vi "Create Palettes for VIs in Folder.vi"(5 "Create palettes for LLBs (F)":bool, 6 "Filter Options":T1={"Exclude Dir Name pattern(s)"="^_", "Exclude LLB Name pattern(s)"="^_", "Exclude VI Name pattern(s)"="^_"}, 7 "Palette Icon":picture, 8 "error in":errorcluster, 9 "Save sub-palettes in sub-folders (F)":bool, 10 "Folder or LLB Path":path, 11 "Palette File Path (empty)":path) -> (0 "error out":errorcluster, 2 "All Palette File Paths":path[](array[path]), 3 "Palette File Path out":path)   [LabVIEW 2014, in "VIHelpeksAPI.lvlib"]
doc: "The VI creates palette files for VIs in a folder. It creates a palette for every sub-folder and LLB beneath the given folder recursively.\n\n<b>Palette icons</b>\nFor the given folder and all sub-folders beneath it, the VI looks for an image file to use as an icon for the respective palette. A folder's icon file can be one of the following:\n(1) A file with the same name as the folder and a <b>.png</b> extension that resides in the folder's parent directory.\n(2) A file with the <b>dir_icon.png</b> name that resides inside the folder itself.\nIf neither of these icon files is found, a default icon is applied to the respective palette.\nThe icon of the top-level palette can be defined explicitly in the <b>Palette Icon</b> input terminal.\n\n\n::: VI Helpeks :::\nCopyright (c) 2000-2026 Konstantin Shifershteyn. All rights reserved."
uses:
  VIHelpeksAPI.lvlib
panel:
  # "VI Helpeks\nCopyright (c) 2012-2026 Konstantin Shifershteyn"
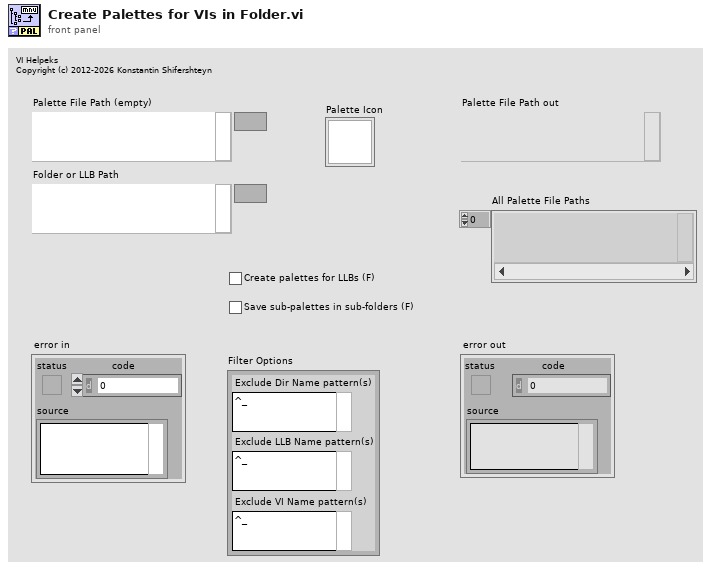
[diagram p1: front panel]
types:
  T1 = cluster{"Exclude Dir Name pattern(s)":string, "Exclude LLB Name pattern(s)":string, "Exclude VI Name pattern(s)":string}
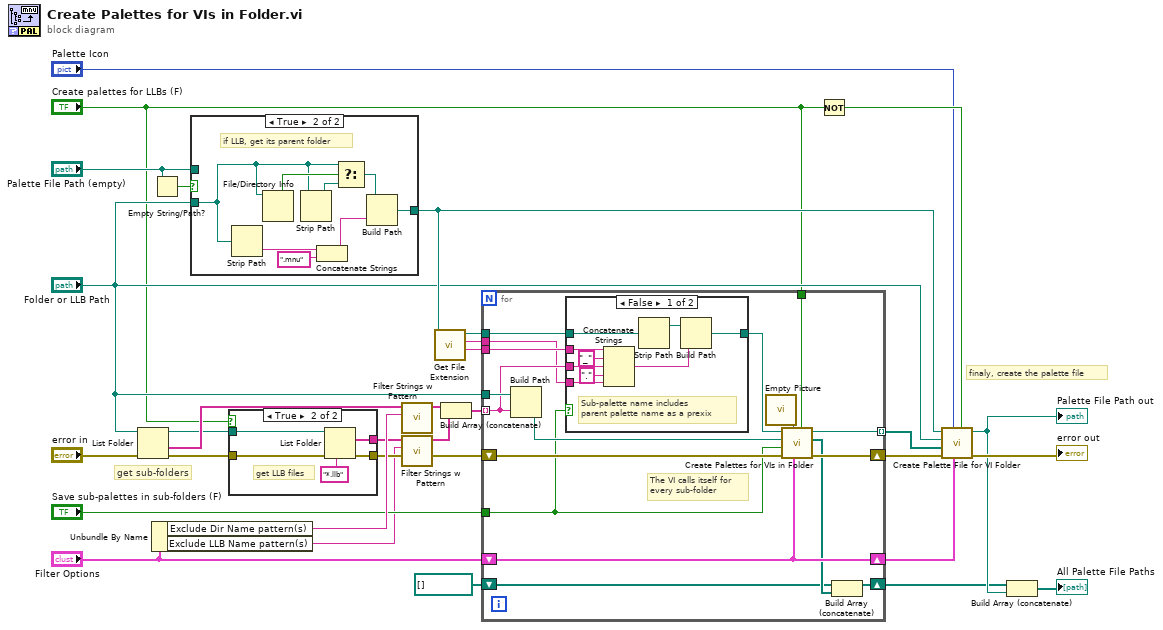
[diagram p0: block diagram]
diagram:
  # "finaly, create the palette file"
  # "get sub-folders"
  n1 = List Folder(path="Folder or LLB Path", error in="error in") -> (path out=w10:path, folder names=w28:string[], error out=w18:errorcluster)  [unwired: 2 in, 1 out]
  n2 = Empty String/Path?(string/path="Palette File Path (empty)") -> (empty?=w25:bool)
  n3 = Unbundle By Name("Filter Options") -> ("Exclude Dir Name pattern(s)"=w27:string, "Exclude LLB Name pattern(s)"=w14:string)
  n4 = case shown="True" w25 {
    tunnel: [w32 w40] -> w23
    tunnel: "Folder or LLB Path" -> [_ w34]
    tunnel: "Palette File Path (empty)" -> [w32 _]
    frame False {
    }
    frame True {
      # "if LLB, get its parent folder"
      n5 = Strip Path(path=w34) -> (name=w33:string)  [unwired: 1 out]
      n6 = File/Directory Info(path=w34) -> (directory=w37:bool)  [unwired: 1 in, 6 out]
      n7 = Strip Path(path=w34) -> (stripped path=w36:path)  [unwired: 1 out]
      n8 = Concatenate Strings(w33, ".mnu" ("string")) -> (w38:string)
      n9 = Select(t=w34, s=w37, f=w36) -> (s? t:f=w35:path)
      n10 = Build Path(base path=w35, name or relative path=w38) -> (appended path=w40:path)
    }
  }
  n11 = case shown="True" "Create palettes for LLBs (F)" {
    tunnel: w18 -> [w41 w45]
    tunnel: [w41 w44] -> w17
    tunnel: w10 -> [_ w43]
    tunnel: [_ w42] -> w15
    frame False {
    }
    frame True {
      # "get LLB files"
      n12 = List Folder(path=w43, pattern="*.llb", error in=w45) -> (filenames=w42:string[], error out=w44:errorcluster)  [unwired: 1 in, 2 out]
    }
  }
  n13 = call "Filter Strings w Pattern.vi"("Exclude pattern(s) (^_)"=w27, "Array in"=w28) -> ("Array out"=w13:string[])  [unwired: 9 in]
  n14 = call "Filter Strings w Pattern.vi"("Exclude pattern(s) (^_)"=w14, "Array in"=w15) -> ("Array out"=w12:string[])  [unwired: 9 in]
  n15 = call <vilib>:"Get File Extension.vi"("file"=w23) -> ("filename without extension"=w22:string, "lowercase file extension"=w21:string, "dup file"=w20:path)  [unwired: 7 in, 1 out]
  n16 = Build Array (concatenate)(w13, w12) -> (w11:string[])
  n17 = for {
    tunnel: "Folder or LLB Path" -> [w63]
    tunnel: w11 -> [w57] mode=indexing
    shift-right: [w61] -> w30
    shift-left: w17 -> [w62]
    tunnel: [w60] -> w8 mode=indexing
    tunnel: w22 -> [w58]
    tunnel: w21 -> [w56]
    tunnel: w20 -> [w55]
    tunnel: "Save sub-palettes in sub-folders (F)" -> [w53]
    shift-right: [w52] -> w9
    shift-left: "Filter Options" -> [w52]
    shift-right: [w49] -> w4
    shift-left: path[] [] -> [w50]
    tunnel: "Create palettes for LLBs (F)" -> [w48]
    # "The VI calls itself for\nevery sub-folder"
    n18 = Build Path(base path=w63, name or relative path=w57) -> (appended path=w59:path)
    n19 = case shown="False" w53 {
      tunnel: w58 -> [w72 _]
      tunnel: w57 -> [w70 _]
      tunnel: w56 -> [w68 _]
      tunnel: w55 -> [w67 _]
      tunnel: [w64 _] -> w54
      frame False {
        # "Sub-palette name includes\nparent palette name as a prexix"
        n20 = Concatenate Strings(w72, "_" ("string"), w70, "." ("string"), w68) -> (w65:string)
        n21 = Strip Path(path=w67) -> (stripped path=w66:path)  [unwired: 1 out]
        n22 = Build Path(base path=w66, name or relative path=w65) -> (appended path=w64:path)
      }
      frame True {
      }
    }
    n23 = call "Empty Picture"() -> ("empty picture"=w47:picture)
    n24 = call "Create Palettes for VIs in Folder.vi"("Create palettes for LLBs (F)"=w48, "Filter Options"=w52, "Palette Icon"=w47, "error in"=w62, "Save sub-palettes in sub-folders (F)"=w53, "Folder or LLB Path"=w59, "Palette File Path (empty)"=w54) -> ("error out"=w61:errorcluster, "All Palette File Paths"=w51:path[], "Palette File Path out"=w60:path)  [unwired: 2 in]
    n25 = Build Array (concatenate)(w50, w51) -> (w49:path[])
  }
  n26 = Not(x="Create palettes for LLBs (F)") -> (.not. x?=w2:bool)
  n27 = call "Create Palette File for VI Folder.vi"("Include VIs in LLBs (T)"=w2, "Filter Options"=w9, "Palette Icon"="Palette Icon", "error in"=w30, "sub-palettes"=w8, "Directory Path"="Folder or LLB Path", "Palette File in"=w23) -> ("error out"=→"error out":errorcluster, "dup Palette File"=w7:path)  [unwired: 2 in, 1 out]
  "Palette File Path out" <- w7
  n28 = Build Array (concatenate)(w4, w7) -> (→"All Palette File Paths":path[])
